vi "Date & Time.vi"() -> (3 "String":string)   [LabVIEW 2026]
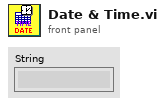
[diagram p1: front panel]
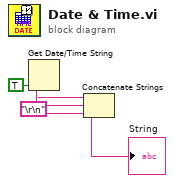
[diagram p0: block diagram]
diagram:
  n1 = Get Date/Time String(want seconds? (F)=TRUE) -> (date string=w2:string, time string=w3:string)  [unwired: 2 in]
  n2 = Concatenate Strings(w2, "\r\n", w3) -> (→"String":string)
